vi "Measurement UI.vi"() -> ()   [LabVIEW 2025, in "Example Plugin UI.lvlib"]
uses:
  Example Plugin UI.lvlib
  <vilib>/gRPC/LabVIEW gRPC Library/Shared/grpcId.ctl
  OOB gRPC Client/RPC Messages/hwval_GenericRequest.ctl
  OOB gRPC Client/RPC Messages/hwval_BoolRequest.ctl
  OOB gRPC Client/RPC Messages/hwval_ExportRequest.ctl
  <vilib>/gRPC/LabVIEW gRPC Library/grpc-lvsupport-release.lvlib
  OOB gRPC Client/OOB gRPC Client.lvlib
panel:
  out "Connection":bool
  out "Double (Loopback)":dbl
  out "String (Loopback)":string
  in  "Send String":bool
  in  "String":string
  in  "Double":dbl
  in  "Send Double":bool
  in  "Export File Type":string(combo)="RAW"
  out "Status":string
  out "Measurement Logic Counter":i32
  out "OOB gRPC Port":i32
  out "Config String (Loopback)":string
  out "Config Number (Loopback)":dbl
  in  "Config String":string="Text"
  in  "Config Number":dbl=1.0
  in  "Export":bool
  in  "PauseResume":bool caption="Pause"
  out "Export (Loopback)":string
  out "PauseResume (Loopback)":bool
  # "Configuration"
  # "Results"
  # "Interactive"
  # "(These controls are not part of the Measurement Confiugration, This way IS doesn't disable and grey them out)"
  # "Status"
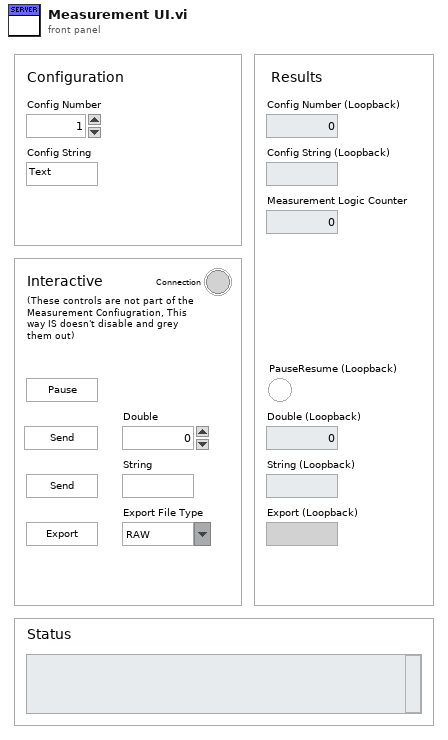
[diagram p1: front panel]
types:
  T1 = typedef "grpc-lvsupport-release.lvlib/grpcId.ctl" = u64
  T2 = typedef "OOB gRPC Client.lvlib/hwval_GenericRequest.ctl" = cluster{"Command":string, "Payload":u8[]}
  T3 = typedef "OOB gRPC Client.lvlib/hwval_BoolRequest.ctl" = cluster{"BooleanData":bool}
  T4 = typedef "OOB gRPC Client.lvlib/hwval_ExportRequest.ctl" = cluster{"FileType":string}
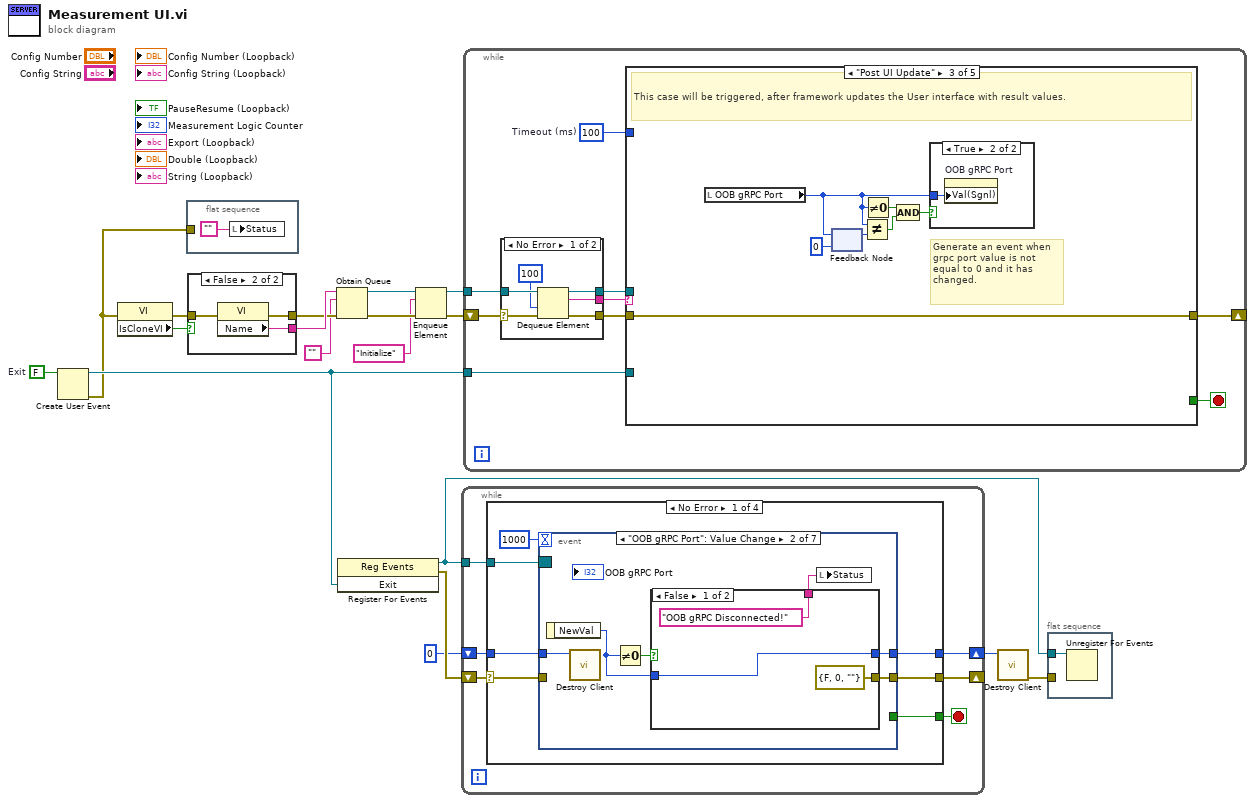
[diagram p0: block diagram]
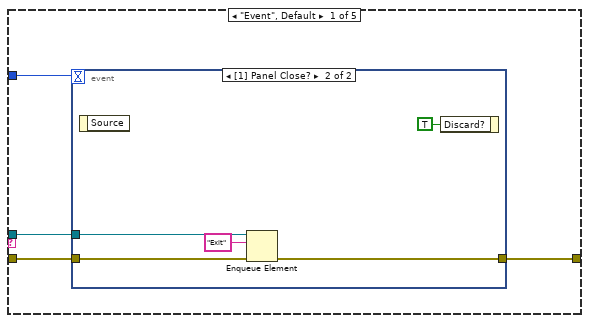
[diagram p2: hidden frame]
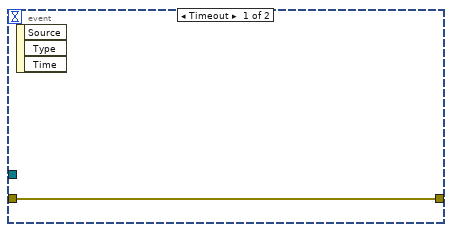
[diagram p3: hidden frame]
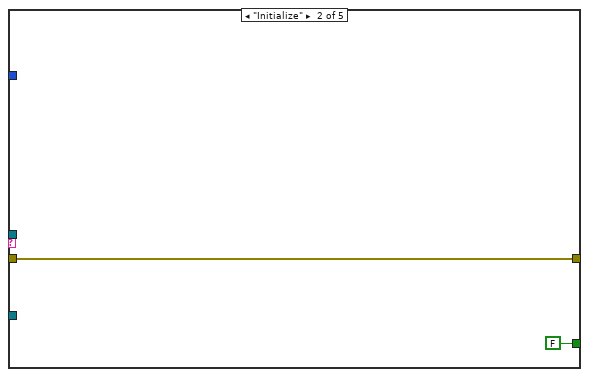
[diagram p4: hidden frame]
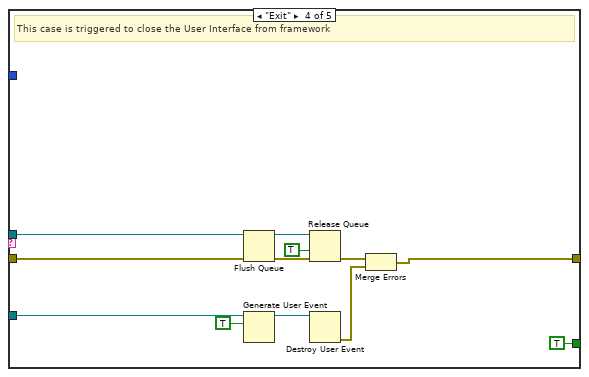
[diagram p6: hidden frame]
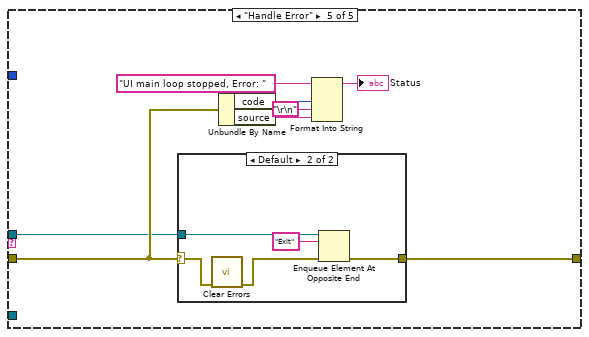
[diagram p7: hidden frame]
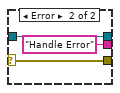
[diagram p9: hidden frame]
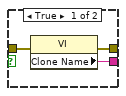
[diagram p10: hidden frame]
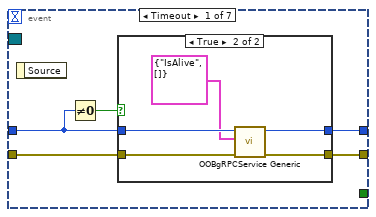
[diagram p11: hidden frame]
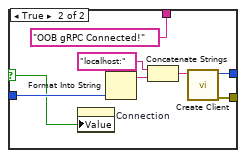
[diagram p13: hidden frame]
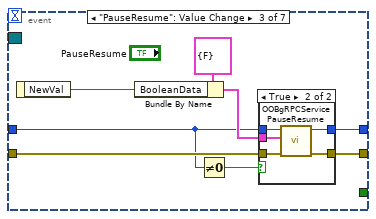
[diagram p14: hidden frame]
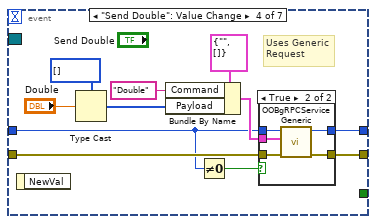
[diagram p16: hidden frame]
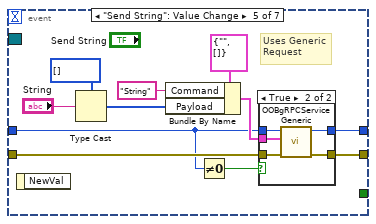
[diagram p18: hidden frame]
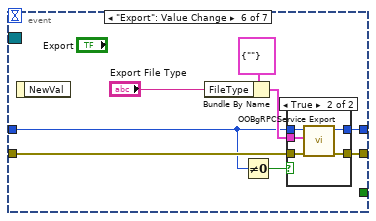
[diagram p20: hidden frame]
diagram:
  w4 = FALSE  # Exit
  n1 = Create User Event(user event datatype=w4) -> (user event=w3:refnum<user-event>, error out=w2:errorcluster)  [unwired: 1 in]
  n2 = property class="VI"(error in=w2) -> (error out=w9:errorcluster, "IsCloneVI"=w14:bool)  [unwired: 1 in, 1 out]
  n3 = flat-sequence {
    tunnel: w2 -> [_]
    frame #0 {
      n4 = local write "Status"("") -> ()
    }
  }
  n5 = case shown="False" w14 {
    tunnel: [w22 w25] -> w13
    tunnel: [w21 w24] -> w18
    tunnel: w9 -> [w20 w23]
    frame True {
      n6 = property class="VI"(error in=w20) -> (error out=w22:errorcluster, "Clone Name"=w21:string)  [unwired: 1 in, 1 out]
    }
    frame False {
      n7 = property class="VI"(error in=w23) -> (error out=w25:errorcluster, "Name"=w24:string)  [unwired: 1 in, 1 out]
    }
  }
  n8 = Obtain Queue(name (unnamed)=w18, element data type="", error in (no error)=w13) -> (queue out=w15:refnum<queue>, error out=w17:errorcluster)  [unwired: 2 in, 1 out]
  n9 = register-events(w3) -> (reference out=w8:refnum<event-registration>, error out=w7:errorcluster)  [unwired: 2 in]
  n10 = Enqueue Element(queue=w15, element="Initialize", error in (no error)=w17) -> (queue out=w10:refnum<queue>, error out=w16:errorcluster)  [unwired: 1 in, 1 out]
  n11 = while {
    tunnel: w8 -> [w28]
    shift-right: [w29] -> _
    shift-left: w7 -> [w31]
    shift-right: [w26] -> w5
    shift-left: T1 0 ("gRPC ID out") -> [w27]
    stop <- w30 stop-if-true
    n12 = case shown="No Error" w31 {
      selector: w31 -> [w36 w138 _ _]
      tunnel: [w33 TRUE w150 w160] -> w30
      tunnel: [w37 w138 errorcluster {"status"=FALSE, "code"=0, "source"=""} ("error IO") errorcluster {"status"=FALSE, "code"=0, "source"=""} ("error IO")] -> w29
      tunnel: w28 -> [w38 _ _ _]
      tunnel: w27 -> [w35 w144 w147 w157]
      tunnel: [w34 w144 w147 w157] -> w26
      frame No Error {
        n13 = event shown="[1] \"OOB gRPC Port\": Value Change" {
          selector: w38 -> [_ _ _ _ _ _ _]
          dyn-events: _ -> [_ _ _ _ _ _ _]
          timeout: 1000 -> [_ _ _ _ _ _ _]
          tunnel: [w42 w56 w74 w92 w110 w125 w134] -> w37
          tunnel: w36 -> [w41 _ w73 w91 w109 w124 w134]
          tunnel: w35 -> [w40 w55 w68 w87 w105 w120 w135]
          tunnel: [w43 w54 w75 w93 w111 w126 w135] -> w34
          tunnel: [_ _ _ _ _ _ w136] -> w33
          event Timeout {
            n14 = event-data() -> ()  [unwired: 1 in, 1 out]
            n15 = Not Equal To 0?(x=w40) -> (x != 0?=w39:bool)
            n16 = case shown="True" w39 {
              tunnel: w40 -> [w45 w50]
              tunnel: [w45 w49] -> w43
              tunnel: [w44 w48] -> w42
              tunnel: w41 -> [w44 w47]
              frame False {
              }
              frame True {
                n17 = call "OOBgRPCService Generic.vi"("error in"=w47, "Request Data"=T2 {"Command"="IsAlive", "Payload"=[]}, "gRPC ID"=w50) -> ("error out"=w48:errorcluster, "gRPC ID out"=w49:T1)  [unwired: 6 in, 1 out]
              }
            }
          }
          event "OOB gRPC Port": Value Change {
            n18 = event-data() -> ("NewVal"=w52:i32)  [unwired: 1 in]
            n19 = call "Destroy Client.vi"("gRPC ID"=w55) -> ()  [unwired: 10 in, 1 out]
            n20 = Not Equal To 0?(x=w52) -> (x != 0?=w53:bool)
            n21 = case shown="False" w53 {
              selector: w53 -> [_ w60]
              tunnel: [errorcluster {"status"=FALSE, "code"=0, "source"=""} ("error out") w67] -> w56
              tunnel: w52 -> [w59 w63]
              tunnel: [w59 w62] -> w54
              tunnel: ["OOB gRPC Disconnected!" ("Status") "OOB gRPC Connected!" ("Status")] -> w51
              frame False {
              }
              frame True {
                n22 = property on="Connection" class="Bool (strict)"("Value"=w60) -> ()  [unwired: 2 in, 2 out]
                n23 = Format Into String(w63) -> (resulting string=w66:string)  [unwired: 3 in, 1 out]
                n24 = Concatenate Strings("localhost:" ("string"), w66) -> (w64:string)
                n25 = call "Create Client.vi"("address"=w64) -> ("error out"=w67:errorcluster, "gRPC ID Out"=w62:T1)  [unwired: 9 in]
              }
            }
            n26 = local write "Status"(w51) -> ()
          }
          event "PauseResume": Value Change {
            n27 = event-data() -> ("NewVal"=w70:bool)  [unwired: 1 in]
            n28 = Bundle By Name(cluster=T3 {"BooleanData"=FALSE} ("Request Data"), "BooleanData"=w70) -> (w71:T3)
            n29 = Not Equal To 0?(x=w68) -> (x != 0?=w69:bool)
            n30 = case shown="True" w69 {
              tunnel: [w77 w82] -> w75
              tunnel: [w76 w81] -> w74
              tunnel: w68 -> [w77 w80]
              tunnel: w73 -> [w76 w79]
              tunnel: w71 -> [_ w78]
              frame False {
              }
              frame True {
                n31 = call "OOBgRPCService PauseResume.vi"("error in"=w79, "Request Data"=w78, "gRPC ID"=w80) -> ("error out"=w81:errorcluster, "gRPC ID out"=w82:T1)  [unwired: 6 in, 1 out]
              }
            }
          }
          event "Send Double": Value Change {
            # "Uses Generic\nRequest"
            n32 = event-data() -> ()  [unwired: 1 in, 1 out]
            n33 = Type Cast(type=u8[] [] ("Payload"), x="Double") -> (*(type *) &x=w83:u8[])
            n34 = Bundle By Name(cluster=T2 {"Command"="", "Payload"=[]} ("Request Data"), "Command"="Double", "Payload"=w83) -> (w89:T2)
            n35 = Not Equal To 0?(x=w87) -> (x != 0?=w88:bool)
            n36 = case shown="True" w88 {
              tunnel: [w95 w100] -> w93
              tunnel: [w94 w99] -> w92
              tunnel: w87 -> [w95 w98]
              tunnel: w91 -> [w94 w97]
              tunnel: w89 -> [_ w96]
              frame False {
              }
              frame True {
                n37 = call "OOBgRPCService Generic.vi"("error in"=w97, "Request Data"=w96, "gRPC ID"=w98) -> ("error out"=w99:errorcluster, "gRPC ID out"=w100:T1)  [unwired: 6 in, 1 out]
              }
            }
          }
          event "Send String": Value Change {
            # "Uses Generic\nRequest"
            n38 = event-data() -> ()  [unwired: 1 in, 1 out]
            n39 = Type Cast(type=u8[] [] ("Payload"), x="String") -> (*(type *) &x=w102:u8[])
            n40 = Bundle By Name(cluster=T2 {"Command"="", "Payload"=[]} ("Request Data"), "Command"="String", "Payload"=w102) -> (w107:T2)
            n41 = Not Equal To 0?(x=w105) -> (x != 0?=w106:bool)
            n42 = case shown="True" w106 {
              tunnel: [w113 w118] -> w111
              tunnel: [w112 w117] -> w110
              tunnel: w105 -> [w113 w116]
              tunnel: w109 -> [w112 w115]
              tunnel: w107 -> [_ w114]
              frame False {
              }
              frame True {
                n43 = call "OOBgRPCService Generic.vi"("error in"=w115, "Request Data"=w114, "gRPC ID"=w116) -> ("error out"=w117:errorcluster, "gRPC ID out"=w118:T1)  [unwired: 6 in, 1 out]
              }
            }
          }
          event "Export": Value Change {
            n44 = event-data() -> ()  [unwired: 1 in, 1 out]
            n45 = Bundle By Name(cluster=T4 {"FileType"=""} ("Request Data"), "FileType"="Export File Type") -> (w122:T4)
            n46 = Not Equal To 0?(x=w120) -> (x != 0?=w121:bool)
            n47 = case shown="True" w121 {
              tunnel: [w128 w133] -> w126
              tunnel: [w127 w132] -> w125
              tunnel: w120 -> [w128 w131]
              tunnel: w124 -> [w127 w130]
              tunnel: w122 -> [_ w129]
              frame False {
              }
              frame True {
                n48 = call "OOBgRPCService Export.vi"("error in"=w130, "Request Data"=w129, "gRPC ID"=w131) -> ("error out"=w132:errorcluster, "gRPC ID out"=w133:T1)  [unwired: 6 in, 1 out]
              }
            }
          }
          event User Event {
            n49 = event-data() -> ("Exit"=w136:bool)  [unwired: 1 in]
          }
        }
      }
      frame Default {
        n50 = Wait (ms)(milliseconds to wait=u32 5000) -> ()  [unwired: 1 out]
        n51 = Unbundle By Name(w138) -> ("code"=w143:i32, "source"=w142:string)
        n52 = Format Into String(initial string="OOB gRPC client loop stopped, Error:" ("format string"), w143, "\r\n", w142) -> (resulting string=w139:string)  [unwired: 2 in, 1 out]
        n53 = local write "Status"(w139) -> ()
      }
      frame Error {
        n54 = local read "OOB gRPC Port"() -> (w152:i32)
        n55 = Wait (ms)(milliseconds to wait=u32 2000) -> ()  [unwired: 1 out]
        n56 = Equal?(x=w152, y=-1 ("x")) -> (x = y?=w150:bool)
        n57 = case shown="False" w150 {
          tunnel: w152 -> [w154 _]
          tunnel: ["Reconnecting.." ("Status") "OOB gRPC server side Error.\nMeasrement Logic didn't get the gRPC port from OOB server.\nRestart the plugin." ("Status")] -> w149
          frame False {
            n58 = property on="OOB gRPC Port" class="DigNum (strict)"("Val(Sgnl)"=w154) -> ()  [unwired: 2 in, 2 out]
          }
          frame True {
          }
        }
        n59 = local write "Status"(w149) -> ()
      }
      frame Error {
        n60 = local read "OOB gRPC Port"() -> (w162:i32)
        n61 = Wait (ms)(milliseconds to wait=u32 100) -> ()  [unwired: 1 out]
        n62 = Equal?(x=w162, y=-1 ("x")) -> (x = y?=w160:bool)
        n63 = case shown="False" w160 {
          selector: w160 -> [w163 _]
          tunnel: w162 -> [_ _]
          tunnel: ["OOB gRPC Disconnted!" ("Status") "OOB gRPC server side Error.\nMeasrement Logic didn't get the gRPC port from OOB server.\nRestart the plugin." ("Status")] -> w159
          frame False {
            n64 = property on="OOB gRPC Port" class="DigNum (strict)"("Val(Sgnl)"=0 ("Value (Signaling)")) -> ()  [unwired: 2 in, 2 out]
            "Connection" <- w163
          }
          frame True {
          }
        }
        n65 = local write "Status"(w159) -> ()
      }
    }
  }
  n66 = while {
    shift-right: [w171] -> _
    shift-left: w16 -> [w175]
    tunnel: w10 -> [w169]
    tunnel: w3 -> [w168]
    stop <- w170 stop-if-true
    w167 = 100  # Timeout (ms)
    n67 = case shown="No Error" w175 {
      selector: w175 -> [w227 w228]
      tunnel: [w226 w228] -> w174
      tunnel: w169 -> [w225 w230]
      tunnel: [w224 w230] -> w173
      tunnel: [w223 "Handle Error"] -> w172
      frame No Error {
        n68 = Dequeue Element(queue=w225, timeout in ms (-1)=100 ("Timeout (ms)"), error in (no error)=w227) -> (queue out=w224:refnum<queue>, element=w223:string, error out=w226:errorcluster)  [unwired: 1 out]
      }
      frame Error {
      }
    }
    n69 = case shown="\"Post UI Update\"" w172 {
      tunnel: w174 -> [w178 w186 w194 w207 w211]
      tunnel: w173 -> [w177 _ _ w205 w209]
      tunnel: [w179 w186 w194 w200 w210] -> w171
      tunnel: [_ FALSE _ TRUE _] -> w170
      tunnel: w167 -> [w176 _ _ _ _]
      tunnel: w168 -> [_ _ _ w196 _]
      frame "Event", Default {
        n70 = event shown="[1] Panel Close?" {
          selector: _ -> [_ _]
          dyn-events: _ -> [_ _]
          timeout: w176 -> [_ _]
          tunnel: [w180 w183] -> w179
          tunnel: w178 -> [w180 w184]
          tunnel: w177 -> [_ w182]
          event Timeout {
            n71 = event-data() -> ()  [unwired: 1 in, 3 out]
          }
          event Panel Close? {
            n72 = event-data() -> ()  [unwired: 1 in, 1 out]
            n73 = Enqueue Element(queue=w182, element="Exit" ("Message"), error in (no error)=w184) -> (error out=w183:errorcluster)  [unwired: 1 in, 2 out]
            n74 = event-data("Discard?"=TRUE) -> ()  [unwired: 1 in, 1 out]
          }
        }
      }
      frame "Initialize" {
      }
      frame "Post UI Update" {
        # "Generate an event when grpc port value is not equal to 0 and it has changed."
        # "This case will be triggered, after framework updates the User interface with result values."
        n75 = local read "OOB gRPC Port"() -> (w189:i32)
        n76 = feedback-in #1(w189) -> ()
        n77 = feedback #1(0 ("OOB gRPC Port")) -> (w188:i32)
        n78 = Not Equal?(x=w189, y=w188) -> (x != y?=w190:bool)
        n79 = Not Equal To 0?(x=w189) -> (x != 0?=w192:bool)
        n80 = Compound Arithmetic op=AND(w192, w190) -> (w191:bool)
        n81 = case shown="True" w191 {
          tunnel: w189 -> [_ w195]
          frame False {
          }
          frame True {
            n82 = property on="OOB gRPC Port" class="DigNum (strict)"("Val(Sgnl)"=w195) -> ()  [unwired: 2 in, 2 out]
          }
        }
      }
      frame "Exit" {
        # "This case is triggered to close the User Interface from framework"
        n83 = Flush Queue(queue=w205, error in (no error)=w207) -> (queue out=w204:refnum<queue>, error out=w203:errorcluster)  [unwired: 1 out]
        n84 = Generate User Event(user event=w196, event data cluster=TRUE ("event data")) -> (user event out=w198:refnum<user-event>)  [unwired: 2 in, 1 out]
        n85 = Release Queue(queue=w204, force destroy? (F)=TRUE, error in (no error)=w203) -> (error out=w202:errorcluster)  [unwired: 2 out]
        n86 = Destroy User Event(user event=w198) -> (error out=w197:errorcluster)  [unwired: 1 in]
        n87 = Merge Errors(w202, w197) -> (w200:errorcluster)
      }
      frame "Handle Error" {
        n88 = case shown="Default" w211 {
          selector: w211 -> [w216 w221]
          tunnel: [w216 w220] -> w210
          tunnel: w209 -> [_ w218]
          frame No Error {
          }
          frame Default {
            n89 = call <vilib>:"Clear Errors.vi"("error in (no error)"=w221) -> ("error out"=w219:errorcluster)  [unwired: 5 in, 1 out]
            n90 = Enqueue Element At Opposite End(queue=w218, element="Exit", error in (no error)=w219) -> (error out=w220:errorcluster)  [unwired: 1 in, 2 out]
          }
        }
        n91 = Unbundle By Name(w211) -> ("code"=w215:i32, "source"=w214:string)
        n92 = Format Into String(initial string="UI main loop stopped, Error: " ("format string"), w215, "\r\n", w214) -> (resulting string=→"Status":string)  [unwired: 2 in, 1 out]
      }
    }
  }
  n93 = call "Destroy Client.vi"("gRPC ID"=w5) -> ("error out"=w6:errorcluster)  [unwired: 10 in]
  n94 = flat-sequence {
    tunnel: w8 -> [w231]
    tunnel: w6 -> [_]
    frame #0 {
      n95 = Unregister For Events(event registration refnum=w231) -> ()  [unwired: 1 in, 1 out]
    }
  }
